vi "Time profile.vi"(8 "Base Ex Info":T2, 11 "Time Probability":dbl[][](array[numeric])) -> (0 "Assigned Profile_plus":T1, 3 "Assigned Profile":T3)   [LabVIEW 2018]
panel:
  out "Array":string[](array[string])
  in  "Q array 2":dbl[](array[numeric])
  out "ASCII_Array":string[](array[string])
  out "Level Composition":string[](array[string])
  out "Assigned lvl array":dbl[](array[numeric])
  out "B array":string[](array[string])
  out "Q array":dbl[](array[numeric])
  out "Probability":dbl[](array[numeric])
  out "Level IDX array":i32[](array[numeric])
  out "サイズ":i32
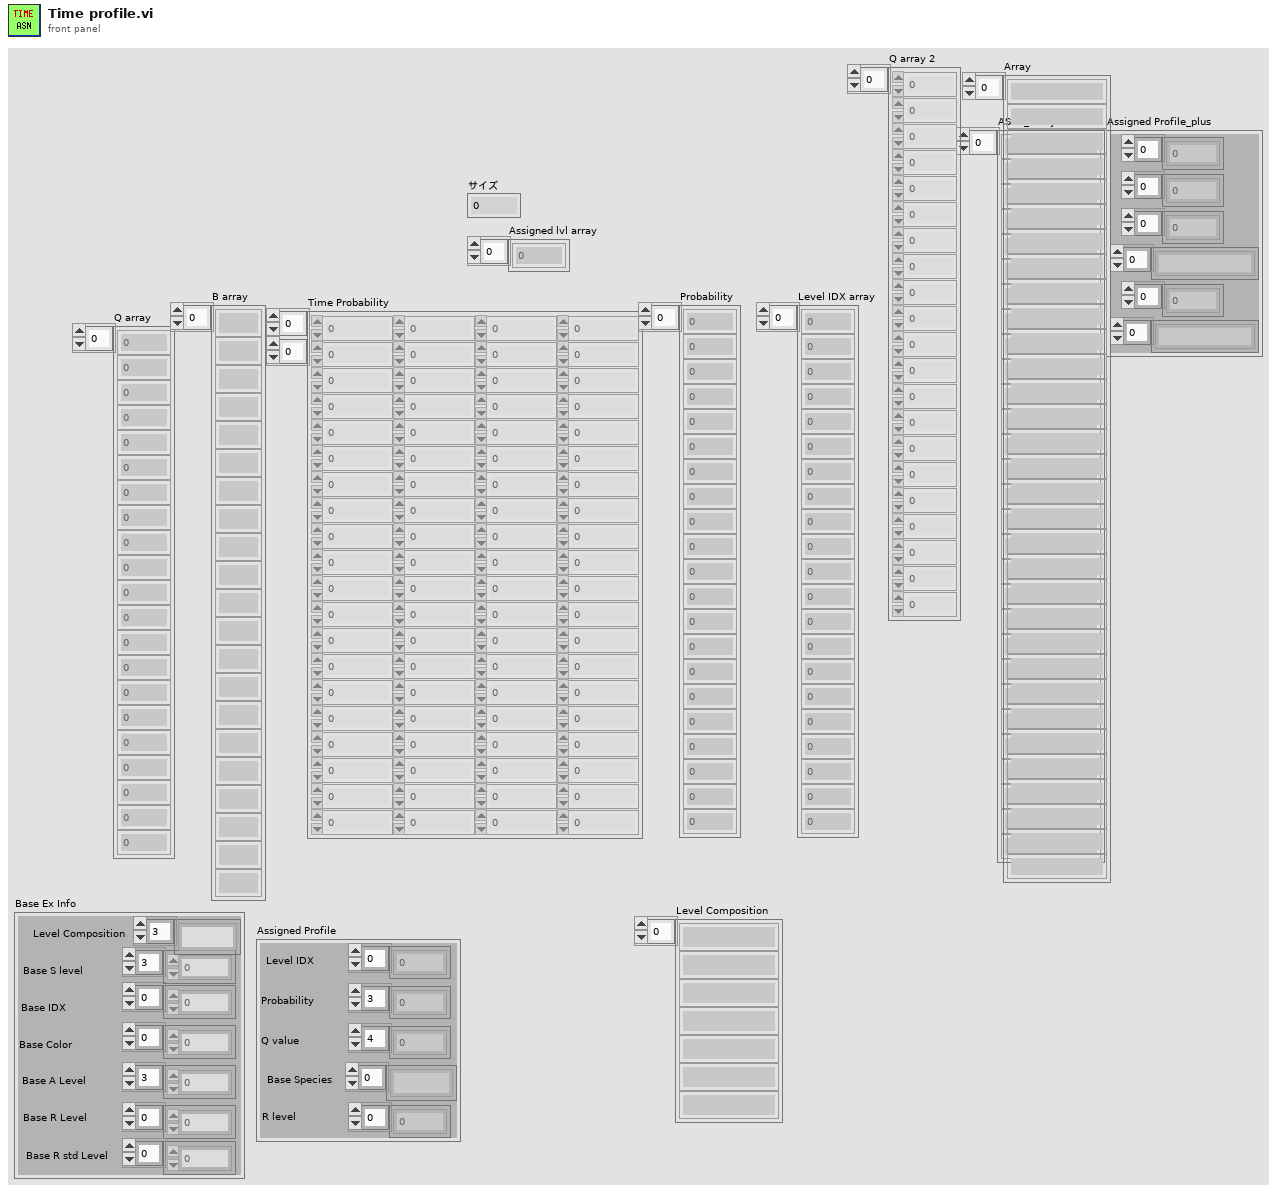
[diagram p1: front panel]
types:
  T1 = cluster{i32[], dbl[], dbl[], string[], dbl[], string[]}
  T2 = cluster{"Level Composition":string[], "Base S level":dbl[], "Base IDX":i32[], "Base Color":u32[], "Base A Level":dbl[], "Base R Level":dbl[], "Base R std Level":dbl[]}
  T3 = cluster{"Level IDX":i32[], "Probability":dbl[], "Q value":dbl[], "Base Species":string[], "R level":dbl[]}
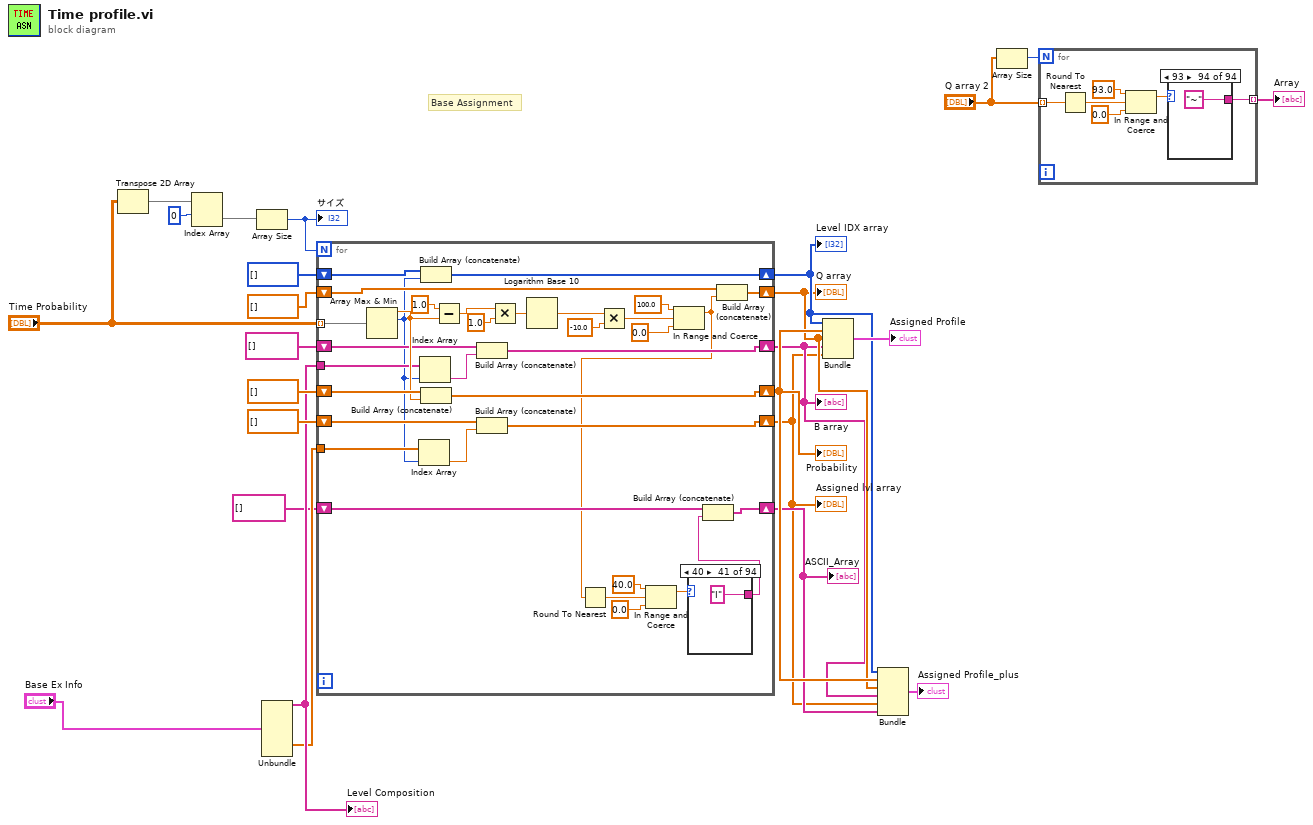
[diagram p0: block diagram]
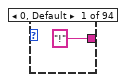
[diagram p2: hidden frame]
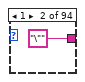
[diagram p3: hidden frame]
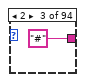
[diagram p4: hidden frame]
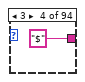
[diagram p5: hidden frame]
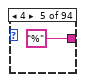
[diagram p6: hidden frame]
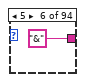
[diagram p7: hidden frame]
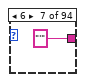
[diagram p8: hidden frame]
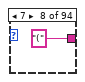
[diagram p9: hidden frame]
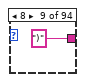
[diagram p10: hidden frame]
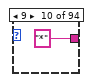
[diagram p11: hidden frame]
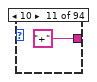
[diagram p12: hidden frame]
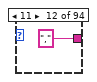
[diagram p13: hidden frame]
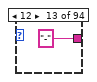
[diagram p14: hidden frame]
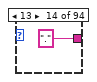
[diagram p15: hidden frame]
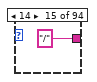
[diagram p16: hidden frame]
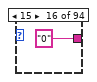
[diagram p17: hidden frame]
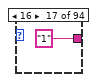
[diagram p18: hidden frame]
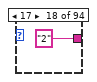
[diagram p19: hidden frame]
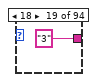
[diagram p20: hidden frame]
diagram:
  # "Base Assignment"
  n1 = Transpose 2D Array(2D array="Time Probability") -> (transposed array=w22:dbl[][])
  n2 = Index Array(array=w22, index (row)=0 ("指標 （行）")) -> (element=w24:dbl[])  [unwired: 1 in]
  n3 = Array Size(array=w24) -> (size(s)=w23:i32)
  "サイズ" <- w23
  n4 = Unbundle("Base Ex Info") -> ("Level Composition"=w14:string[], "Base R Level"=w13:dbl[])  [unwired: 5 out]
  "Level Composition" <- w14
  n5 = for {
    N: w23 -> [_]
    tunnel: "Time Probability" -> [w59] mode=indexing
    shift-right: [w58] -> w10
    shift-left: i32[] [] -> [w57]
    shift-right: [w50] -> w9
    shift-left: dbl[] [] -> [w49]
    shift-right: [w47] -> w8
    shift-left: dbl[] [] -> [w46]
    shift-right: [w42] -> w7
    shift-left: string[] [] -> [w41]
    shift-right: [w40] -> w5
    shift-left: dbl[] [] -> [w39]
    tunnel: w13 -> [w38]
    tunnel: w14 -> [w36]
    shift-right: [w32] -> w6
    shift-left: string[] [] -> [w33]
    n6 = Array Max & Min(array=w59) -> (max value=w48:dbl, max index (indices)=w35:i32)  [unwired: 2 out]
    n7 = Index Array(array=w38, index=w35) -> (element=w37:dbl)
    n8 = Index Array(array=w36, index=w35) -> (element=w34:string)
    n9 = Build Array (concatenate)(w57, w35) -> (w58:i32[])
    n10 = Build Array (concatenate)(w49, w48) -> (w50:dbl[])
    n11 = Subtract(x=1.0, y=w48) -> (x-y=w53:dbl)
    n12 = Build Array (concatenate)(w41, w34) -> (w42:string[])
    n13 = Build Array (concatenate)(w39, w37) -> (w40:dbl[])
    n14 = Multiply(x=w53, y=1.0) -> (x*y=w52:dbl)
    n15 = Logarithm Base 10(1:w52) -> (0:w56:dbl)
    n16 = Multiply(x=w56, y=-10.0) -> (x*y=w45:dbl)
    n17 = In Range and Coerce(upper limit=100.0 ("上限"), x=w45, lower limit=0.0 ("下限")) -> (coerced(x)=w27:dbl)  [unwired: 1 out]
    n18 = Round To Nearest(number=w27) -> (nearest integer value=w29:dbl)
    n19 = In Range and Coerce(upper limit=40.0, x=w29, lower limit=0.0) -> (coerced(x)=w28:dbl)  [unwired: 1 out]
    n20 = case shown="40" w28 {
      tunnel: ["!" "\"" "#" "$" "%" "&" "'" "(" ")" "*" "+" "," "-" "." "/" "0" "1" "2" "3" "4" "5" "6" "7" "8" "9" ":" ";" "<" "=" ">" "?" "@" "A" "B" "C" "D" "E" "F" "G" "H" "I" "J" "K" "L" "M" "N" "O" "P" "Q" ("String") "R" ("String") "S" ("String") "T" ("String") "U" ("String") "V" ("String") "W" ("String") "X" ("String") "Y" ("String") "Z" ("String") "[" ("String") "\\" ("String") "]" ("String") "^" ("String") "_" ("String") "`" ("String") "a" ("String") "b" ("String") "c" ("String") "d" ("String") "e" ("String") "f" ("String") "g" ("String") "h" ("String") "i" ("String") "j" ("String") "k" ("String") "l" ("String") "m" ("String") "n" ("String") "o" ("String") "p" ("String") "q" ("String") "r" ("String") "s" ("String") "t" ("String") "u" ("String") "v" ("String") "w" ("String") "x" ("String") "y" ("String") "z" ("String") "{" ("String") "\t|" ("String") "}" ("String") "~" ("String")] -> w26
      frame 0, Default {
      }
      frame 1 {
      }
      frame 2 {
      }
      frame 3 {
      }
      frame 4 {
      }
      frame 5 {
      }
      frame 6 {
      }
      frame 7 {
      }
      frame 8 {
      }
      frame 9 {
      }
      frame 10 {
      }
      frame 11 {
      }
      frame 12 {
      }
      frame 13 {
      }
      frame 14 {
      }
      frame 15 {
      }
      frame 16 {
      }
      frame 17 {
      }
      frame 18 {
      }
      frame 19 {
      }
      frame 20 {
      }
      frame 21 {
      }
      frame 22 {
      }
      frame 23 {
      }
      frame 24 {
      }
      frame 25 {
      }
      frame 26 {
      }
      frame 27 {
      }
      frame 28 {
      }
      frame 29 {
      }
      frame 30 {
      }
      frame 31 {
      }
      frame 32 {
      }
      frame 33 {
      }
      frame 34 {
      }
      frame 35 {
      }
      frame 36 {
      }
      frame 37 {
      }
      frame 38 {
      }
      frame 39 {
      }
      frame 40 {
      }
      frame 41 {
      }
      frame 42 {
      }
      frame 43 {
      }
      frame 44 {
      }
      frame 45 {
      }
      frame 46 {
      }
      frame 47 {
      }
      frame 48 {
      }
      frame 49 {
      }
      frame 50 {
      }
      frame 51 {
      }
      frame 52 {
      }
      frame 53 {
      }
      frame 54 {
      }
      frame 55 {
      }
      frame 56 {
      }
      frame 57 {
      }
      frame 58 {
      }
      frame 59 {
      }
      frame 60 {
      }
      frame 61 {
      }
      frame 62 {
      }
      frame 63 {
      }
      frame 64 {
      }
      frame 65 {
      }
      frame 66 {
      }
      frame 67 {
      }
      frame 68 {
      }
      frame 69 {
      }
      frame 70 {
      }
      frame 71 {
      }
      frame 72 {
      }
      frame 73 {
      }
      frame 74 {
      }
      frame 75 {
      }
      frame 76 {
      }
      frame 77 {
      }
      frame 78 {
      }
      frame 79 {
      }
      frame 80 {
      }
      frame 81 {
      }
      frame 82 {
      }
      frame 83 {
      }
      frame 84 {
      }
      frame 85 {
      }
      frame 86 {
      }
      frame 87 {
      }
      frame 88 {
      }
      frame 89 {
      }
      frame 90 {
      }
      frame 91 {
      }
      frame 92 {
      }
      frame 93 {
      }
    }
    n21 = Build Array (concatenate)(w33, w26) -> (w32:string[])
    n22 = Build Array (concatenate)(w46, w27) -> (w47:dbl[])
  }
  "Level IDX array" <- w10
  "Probability" <- w9
  "Q array" <- w8
  "B array" <- w7
  "Assigned lvl array" <- w5
  "ASCII_Array" <- w6
  n23 = Bundle(w10, w9, w8, w7, w5) -> (→"Assigned Profile":cluster{i32[], dbl[], dbl[], string[], dbl[]})  [unwired: 1 in]
  n24 = Bundle(w10, w9, w8, w7, w5, w6) -> (→"Assigned Profile_plus":T1)  [unwired: 1 in]
  n25 = Array Size(array="Q array 2") -> (size(s)=w3:i32)
  n26 = for {
    N: w3 -> [_]
    tunnel: "Q array 2" -> [w159] mode=indexing
    tunnel: [w158] -> w1 mode=indexing
    n27 = Round To Nearest(number=w159) -> (nearest integer value=w155:dbl)
    n28 = In Range and Coerce(upper limit=93.0, x=w155, lower limit=0.0) -> (coerced(x)=w154:dbl)  [unwired: 1 out]
    n29 = case shown="93" w154 {
      tunnel: ["!" "\"" "#" "$" "%" "&" "'" "(" ")" "*" "+" "," "-" "." "/" "0" "1" "2" "3" "4" "5" "6" "7" "8" "9" ":" ";" "<" "=" ">" "?" "@" "A" "B" "C" "D" "E" "F" "G" "H" "I" "J" "K" "L" "M" "N" "O" "P" "Q" ("String") "R" ("String") "S" ("String") "T" ("String") "U" ("String") "V" ("String") "W" ("String") "X" ("String") "Y" ("String") "Z" ("String") "[" ("String") "\\" ("String") "]" ("String") "^" ("String") "_" ("String") "`" ("String") "a" ("String") "b" ("String") "c" ("String") "d" ("String") "e" ("String") "f" ("String") "g" ("String") "h" ("String") "i" ("String") "j" ("String") "k" ("String") "l" ("String") "m" ("String") "n" ("String") "o" ("String") "p" ("String") "q" ("String") "r" ("String") "s" ("String") "t" ("String") "u" ("String") "v" ("String") "w" ("String") "x" ("String") "y" ("String") "z" ("String") "{" ("String") "\t|" ("String") "}" ("String") "~" ("String")] -> w158
      frame 0, Default {
      }
      frame 1 {
      }
      frame 2 {
      }
      frame 3 {
      }
      frame 4 {
      }
      frame 5 {
      }
      frame 6 {
      }
      frame 7 {
      }
      frame 8 {
      }
      frame 9 {
      }
      frame 10 {
      }
      frame 11 {
      }
      frame 12 {
      }
      frame 13 {
      }
      frame 14 {
      }
      frame 15 {
      }
      frame 16 {
      }
      frame 17 {
      }
      frame 18 {
      }
      frame 19 {
      }
      frame 20 {
      }
      frame 21 {
      }
      frame 22 {
      }
      frame 23 {
      }
      frame 24 {
      }
      frame 25 {
      }
      frame 26 {
      }
      frame 27 {
      }
      frame 28 {
      }
      frame 29 {
      }
      frame 30 {
      }
      frame 31 {
      }
      frame 32 {
      }
      frame 33 {
      }
      frame 34 {
      }
      frame 35 {
      }
      frame 36 {
      }
      frame 37 {
      }
      frame 38 {
      }
      frame 39 {
      }
      frame 40 {
      }
      frame 41 {
      }
      frame 42 {
      }
      frame 43 {
      }
      frame 44 {
      }
      frame 45 {
      }
      frame 46 {
      }
      frame 47 {
      }
      frame 48 {
      }
      frame 49 {
      }
      frame 50 {
      }
      frame 51 {
      }
      frame 52 {
      }
      frame 53 {
      }
      frame 54 {
      }
      frame 55 {
      }
      frame 56 {
      }
      frame 57 {
      }
      frame 58 {
      }
      frame 59 {
      }
      frame 60 {
      }
      frame 61 {
      }
      frame 62 {
      }
      frame 63 {
      }
      frame 64 {
      }
      frame 65 {
      }
      frame 66 {
      }
      frame 67 {
      }
      frame 68 {
      }
      frame 69 {
      }
      frame 70 {
      }
      frame 71 {
      }
      frame 72 {
      }
      frame 73 {
      }
      frame 74 {
      }
      frame 75 {
      }
      frame 76 {
      }
      frame 77 {
      }
      frame 78 {
      }
      frame 79 {
      }
      frame 80 {
      }
      frame 81 {
      }
      frame 82 {
      }
      frame 83 {
      }
      frame 84 {
      }
      frame 85 {
      }
      frame 86 {
      }
      frame 87 {
      }
      frame 88 {
      }
      frame 89 {
      }
      frame 90 {
      }
      frame 91 {
      }
      frame 92 {
      }
      frame 93 {
      }
    }
  }
  "Array" <- w1
